vi "TP.vi"(10 "Time":i32, 11 "Trigger":bool) -> (2 "ET 4":i32, 3 "Q 4":bool)   [LabVIEW 2020]
uses:
  0fadf32d-e5bc-4af1-a2c4-0be75654e99c.vi
panel:
  out "Time memory":i32
  out "Memory bit 2":bool
  out "Memory bit 1":bool
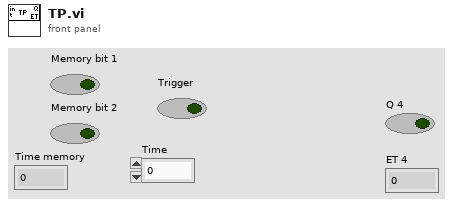
[diagram p1: front panel]
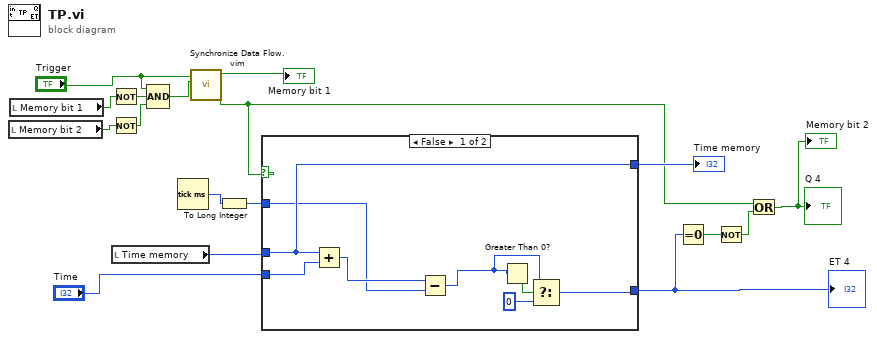
[diagram p0: block diagram]
diagram:
  n1 = local read "Memory bit 2"() -> (w5:bool)
  n2 = local read "Memory bit 1"() -> (w6:bool)
  n3 = Not(x=w6) -> (.not. x?=w17:bool)
  n4 = Not(x=w5) -> (.not. x?=w10:bool)
  n5 = local read "Time memory"() -> (w7:i32)
  n6 = Compound Arithmetic op=AND("Trigger", w17, w10) -> (w2:bool)
  n7 = Tick Count (ms)() -> (millisecond timer value=w16:u32)
  n8 = call "Synchronize Data Flow.vim"("input 2"=w2, "input 1"="Trigger") -> ("output 2"=w1:bool, "output 1"=→"Memory bit 1":bool)  [unwired: 2 in, 2 out]
  n9 = To Long Integer(number=w16) -> (32bit integer=w15:i32)
  n10 = case shown="False" w1 {
    tunnel: w15 -> [w19 w27]
    tunnel: [w20 w27] -> w9
    tunnel: w7 -> [w20 _]
    tunnel: "Time" -> [w21 w26]
    tunnel: [w18 w26] -> w12
    frame False {
      n11 = Add(x=w20, y=w21) -> (x+y=w25:i32)
      n12 = Subtract(x=w25, y=w19) -> (x-y=w23:i32)
      n13 = Greater Than 0?(x=w23) -> (x > 0?=w24:bool)
      n14 = Select(t=w23, s=w24, f=0) -> (s? t:f=w18:i32)
    }
    frame True {
    }
  }
  "ET 4" <- w12
  "Time memory" <- w9
  n15 = Equal To 0?(x=w12) -> (x = 0?=w11:bool)
  n16 = Not(x=w11) -> (.not. x?=w14:bool)
  n17 = Or(x=w1, y=w14) -> (x .or. y?=→"Q 4" →"Memory bit 2":bool)
